vi "CoolProp.vi"(6 "Fluid":string="Water", 7 "Output":string="T", 8 "Value2":dbl=1.0, 10 "Value1":dbl=400.0) -> (0 "error_message":string, 3 "Return Value":dbl=416.75835925510785)   [LabVIEW 2019]
uses:
  CoolProp.dll
panel:
  in  "Input2":string
  in  "Input1":string
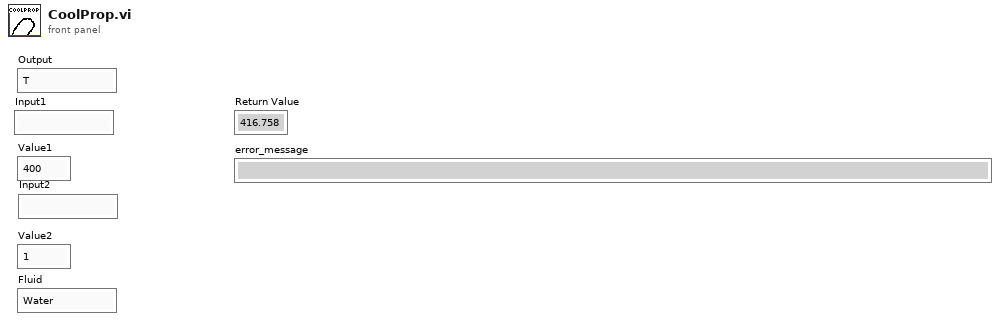
[diagram p1: front panel]
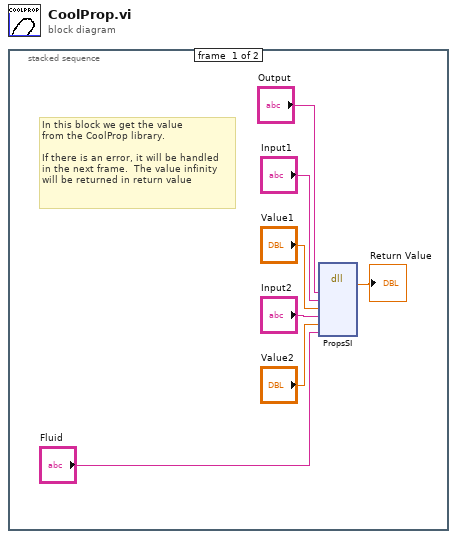
[diagram p0: block diagram]
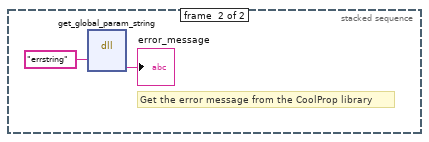
[diagram p2: hidden frame]
diagram:
  n1 = stacked-sequence {
    frame #0 {
      # "In this block we get the value\nfrom the CoolProp library.\n\nIf there is an error, it will be handled\nin the next frame.  The value infinity \nwill be returned in return value"
      n2 = dll-call lib="\\\\VBOXSVR\\passthrough/CoolProp.dll" fn="PropsSI"("Output"="Output", "Input1"="Input1", "Value1"="Value1", "Input2"="Input2", "Value2"="Value2", "Fluid"="Fluid") -> ("OutputValue"=→"Return Value":dbl)  [unwired: 9 in, 2 out]
    }
    frame #1 {
      # "Get the error message from the CoolProp library"
      n3 = dll-call lib="\\\\VBOXSVR\\passthrough/CoolProp.dll" fn="get_global_param_string"("param"="errstring") -> ("error_message"=→"error_message":string)  [unwired: 4 in, 4 out]
    }
  }
